vi "Activida 1 Interfaz LABVIEW.vi"() -> ()   [LabVIEW 2026]
panel:
  in  "stop":bool
  out "Frio":bool
  out "Caliente":bool
  out "Celcius":dbl(slide) scale=0.0..100.0
  out "Kelvin":dbl(slide) scale=273.0..373.0
  out "Farenheit":dbl(slide) scale=32.0..212.0
  in  "Slider":dbl(slide) scale=-20.0..100.0
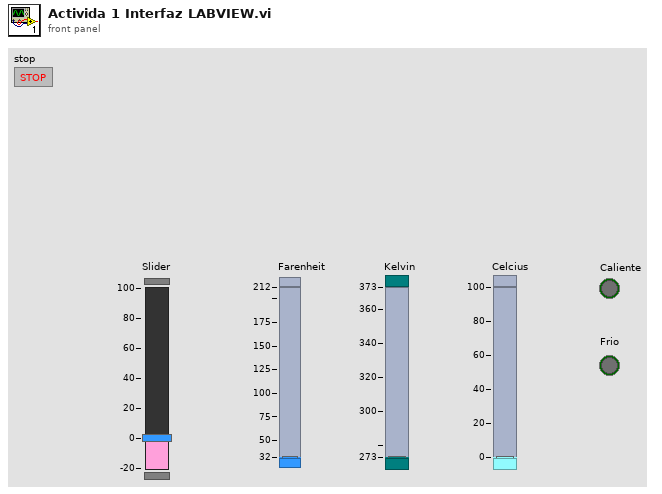
[diagram p1: front panel]
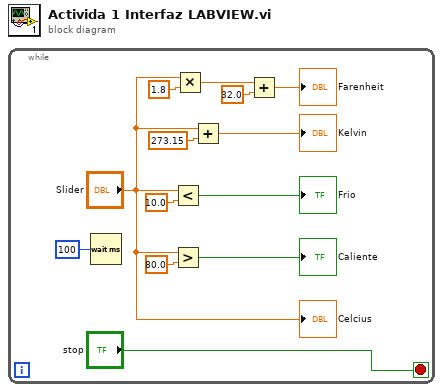
[diagram p0: block diagram]
diagram:
  n1 = while {
    stop <- "stop" stop-if-true
    n2 = Wait (ms)(milliseconds to wait=u32 100) -> ()  [unwired: 1 out]
    n3 = Less?(x="Slider", y=10.0) -> (x < y?=→"Frio":bool)
    n4 = Greater?(x="Slider", y=80.0) -> (0:→"Caliente":bool)
    n5 = Multiply(x="Slider", y=1.8) -> (x*y=w11:dbl)
    n6 = Add(x="Slider", y=273.15) -> (x+y=→"Kelvin":dbl)
    n7 = Add(x=w11, y=32.0) -> (x+y=→"Farenheit":dbl)
    "Celcius" <- "Slider"
  }
